vi "EJERCICIO _1_FOR_TEMPORIZADOR.vi"() -> ()   [LabVIEW 2026]
panel:
  out "INDICADOR":i16
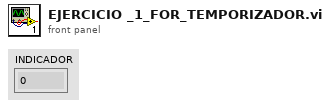
[diagram p1: front panel]
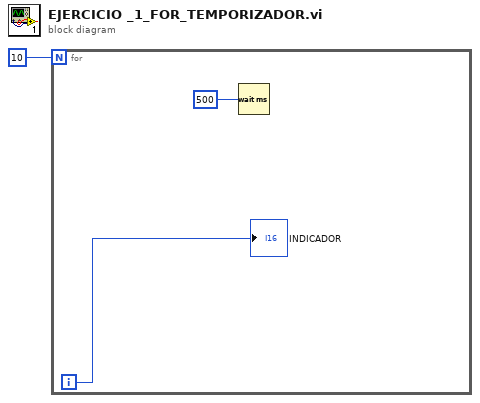
[diagram p0: block diagram]
diagram:
  n1 = for {
    N: 10 -> [_]
    i -> [w3]
    n2 = Wait (ms)(milliseconds to wait=500) -> ()  [unwired: 1 out]
    "INDICADOR" <- w3
  }
